vi "Stock Catalogue.vi"() -> (2 "sectors":string[](array[string]), 3 "stocks":T1[](array[typedef]))   [LabVIEW 2020, in "Full Featured MCP Server.lvlib"]
doc: "The stocks of the simulated market, one row per stock. Edit the constant to change the market: name, sector (index into sectors), quality (-1 weak, 0 average, 1 strong: leans news and story endings), start price in euros, drift (average log return per second: the trend), volatility (random move per second), beta (how strongly the stock follows the market mood), jumpiness (chance per second of an unusually big move) and the description the assistant reads."
uses:
  Full Featured MCP Server.lvlib
  Stock Entry.ctl
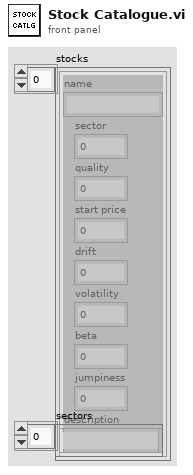
[diagram p1: front panel]
types:
  T1 = typedef "Full Featured MCP Server.lvlib/Stock Entry.ctl" = cluster{"name":string, "sector":i32, "quality":i32, "start price":dbl, "drift":dbl, "volatility":dbl, "beta":dbl, "jumpiness":dbl, "description":string}
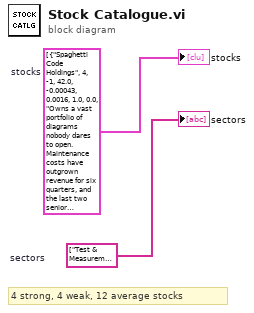
[diagram p0: block diagram]
diagram:
  w2 = string[] ["Test & Measurement Hardware", "Real-Time & FPGA", "Software Architecture", "Data & Logging", "Legacy Code"]  # sectors
  w1 = T1[] [{"name"="Spaghetti Code Holdings", "sector"=4, "quality"=-1, "start price"=42.0, "drift"=-0.00043, "volatility"=0.0016, "beta"=1.0, "jumpiness"=0.0, "description"="Owns a vast portfolio of diagrams nobody dares to open. Maintenance costs have outgrown revenue for six quarters, and the last two senior developers left without writing documentation."}, {"name"="Broken Arrow Technologies", "sector"=0, "quality"=0, "start price"=18.0, "drift"=2e-05, "volatility"=0.0025, "beta"=1.3, "jumpiness"=0.01, "description"="Sells fixes for run arrows it sometimes breaks itself. Every release either doubles the customer base or triggers a recall; analysts have stopped forecasting it."}, {"name"="Race Condition Capital", "sector"=1, "quality"=0, "start price"=95.0, "drift"=-2e-05, "volatility"=0.0025, "beta"=1.5, "jumpiness"=0.015, "description"="A fund whose results depend on which thread gets there first. Brilliant quarters and dreadful ones alternate without a visible pattern."}, {"name"="Coercion Dot Commodities", "sector"=3, "quality"=0, "start price"=12.0, "drift"=0.0, "volatility"=0.0018, "beta"=0.8, "jumpiness"=0.0, "description"="Trades little red dots in bulk. Margins are thin and occasionally lose precision, but the warehouses are full and demand never quite goes away."}, {"name"="Infinite While Loop Inc.", "sector"=4, "quality"=-1, "start price"=27.0, "drift"=-0.00048, "volatility"=0.0018, "beta"=1.1, "jumpiness"=0.01, "description"="Promises to finish the product in the next iteration. Cash burn is constant, the stop condition was never wired, and the main investor has asked for his money back."}, {"name"="PXI Chassis Real Estate", "sector"=0, "quality"=0, "start price"=310.0, "drift"=2e-05, "volatility"=0.0009, "beta"=0.6, "jumpiness"=0.0, "description"="Rents out slots. Occupancy is solid, but growth depends on how many new chassis the industry builds this year."}, {"name"="FlexLogger Log Files", "sector"=3, "quality"=1, "start price"=64.0, "drift"=0.00038, "volatility"=0.0014, "beta"=0.9, "jumpiness"=0.0, "description"="Stores what everybody else measures. Renewal rate above 95 percent, storage costs falling every quarter, and a waiting list for the new cloud tier. The founder still answers support tickets himself."}, {"name"="VeriStand Simulation Systems", "sector"=1, "quality"=0, "start price"=140.0, "drift"=2e-05, "volatility"=0.0018, "beta"=1.0, "jumpiness"=0.0, "description"="Simulates everything except its own sales pipeline. Solid engineering, long project cycles, and revenue that arrives late but usually arrives."}, {"name"="TestStand Sequence Sprawl", "sector"=2, "quality"=0, "start price"=88.0, "drift"=1e-05, "volatility"=0.0009, "beta"=0.5, "jumpiness"=0.0, "description"="Ugly architecture, reliable income: half the industry's test racks run its sequences. Growth is flat, the dividend is not in danger, and nobody is excited."}, {"name"="DAQmx Task Force", "sector"=0, "quality"=1, "start price"=230.0, "drift"=0.00036, "volatility"=0.0013, "beta"=1.0, "jumpiness"=0.0, "description"="Create, start, read, clear: four calls and the job is done. Order backlog at a record, two new factories on schedule, margins rising. Critics say the price already knows all that."}, {"name"="cRIO Real-Time Jitter", "sector"=1, "quality"=0, "start price"=55.0, "drift"=-2e-05, "volatility"=0.0023, "beta"=1.4, "jumpiness"=0.01, "description"="Deterministic on paper, nervous in practice. Wins big contracts and loses them again over delivery dates; the share price twitches accordingly."}, {"name"="FPGA Compile Time Waits", "sector"=1, "quality"=0, "start price"=35.0, "drift"=0.0, "volatility"=0.0005, "beta"=0.2, "jumpiness"=0.0, "description"="Sells patience by the hour. Nothing happens for long stretches, then a build finishes and the books look exactly as before."}, {"name"="Shift Register Savings", "sector"=2, "quality"=1, "start price"=120.0, "drift"=0.0004, "volatility"=0.0011, "beta"=0.7, "jumpiness"=0.0, "description"="Keeps state where it belongs. Twelve quarters of rising recurring revenue, no debt, and a customer list that renews without being asked."}, {"name"="Unbundled Cluster Mess", "sector"=3, "quality"=-1, "start price"=23.0, "drift"=-0.00041, "volatility"=0.0018, "beta"=1.1, "jumpiness"=0.005, "description"="Took a tidy business apart and cannot find the pieces. Three divisions report in three formats, two of them at a loss; the new CFO is the fourth in two years. Slogan: Everything in its place."}, {"name"="Polymorphic Selector Group", "sector"=2, "quality"=0, "start price"=76.0, "drift"=2e-05, "volatility"=0.0018, "beta"=1.0, "jumpiness"=0.0, "description"="Has a product for every data type and a different strategy for each. Some instances earn well, others are quietly being deprecated."}, {"name"="SubVI Reentrancy Labs", "sector"=1, "quality"=1, "start price"=180.0, "drift"=0.00041, "volatility"=0.0016, "beta"=1.2, "jumpiness"=0.005, "description"="Does many things at once without mixing them up. Patent portfolio growing, licence income up by a third, and the big integrators are standardising on its clones. Spends heavily on research."}, {"name"="Global Variable Chaos", "sector"=4, "quality"=-1, "start price"=9.5, "drift"=-0.00051, "volatility"=0.0021, "beta"=1.2, "jumpiness"=0.01, "description"="Everyone can write to everything, including the balance sheet. Third restatement of earnings in two years; the auditor resigned in spring."}, {"name"="Local Variable Abuse Co.", "sector"=4, "quality"=0, "start price"=48.0, "drift"=-3e-05, "volatility"=0.0018, "beta"=1.0, "jumpiness"=0.005, "description"="Takes shortcuts and mostly gets away with it. Earnings are decent, but every few months a hidden side effect shows up in the accounts."}, {"name"="Flat Sequence Films", "sector"=4, "quality"=0, "start price"=15.0, "drift"=1e-05, "volatility"=0.0013, "beta"=0.6, "jumpiness"=0.0, "description"="Tells its stories strictly frame by frame. A loyal audience, modest budgets, and no ambition to do two things at the same time."}, {"name"="Stacked Sequence Mysteries", "sector"=4, "quality"=0, "start price"=400.0, "drift"=0.0, "volatility"=0.0006, "beta"=0.3, "jumpiness"=0.0, "description"="Hides its business in frames nobody sees at once. What is visible looks fine; analysts disagree about the rest and mostly ignore the stock."}]  # stocks
  # "4 strong, 4 weak, 12 average stocks"
  "stocks" <- w1
  "sectors" <- w2
